vi "Encode String.vi"(7 "Prepend BOM (F)":bool, 8 "error in":errorcluster, 9 "Output Encoding (UTF-16LE)":T1=enum."UTF-16LE", 10 "Input Encoding (ANSI)":T1, 11 "String in":string) -> (0 "error out":errorcluster, 3 "String out":string)   [LabVIEW 2020, in "G-Unicode.lvlib"]
doc: "Encodes the text in <b>String</b> with the encoding specified by <b>Output Encoding</b>. The input String encoding is defined by <b>Input Encoding</b>. If Output Encoding is unicode (UTF-8 or UTF-16), the corresponding Byte Order Mark (BOM) can be prepended by setting <b>Prepend BOM</b> to TRUE.\n\nIf the input string encoding isn't known, Input Encoding can be set to Unknown to try and automatically detect the encoding method. Note that automatic encoding detection isn't 100% accurate, and it is recommended to set the encoding explicitly if it is known.\n\nSupported input/output encodings:\nANSI\nUTF-8\nUTF-16LE\nUTF-16BE"
uses:
  G-Unicode.lvlib
  Controls/String Encoding.ctl
  Private/Conversion/Polymorphic VIs/Text to UTF-8 (LabVIEW String).vi
  Private/Conversion/Polymorphic VIs/UTF-8 to Text (LabVIEW String).vi
  SubVIs/Byte Order Marks.vi
  Detect BOM.vi
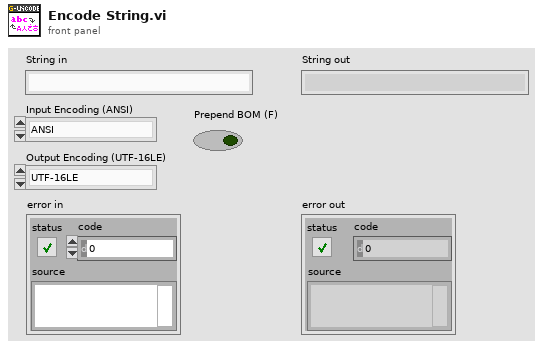
[diagram p1: front panel]
types:
  T1 = typedef "G-Unicode.lvlib/String Encoding.ctl" = enum16{"ANSI", "UTF-8", "UTF-16LE", "UTF-16BE", "Unknown"}
  T2 = typedef "G-Unicode.lvlib/Encoded UTF-8 String.ctl" = string
  T3 = typedef "G-Unicode.lvlib/Encoded UTF-16LE String.ctl" = string
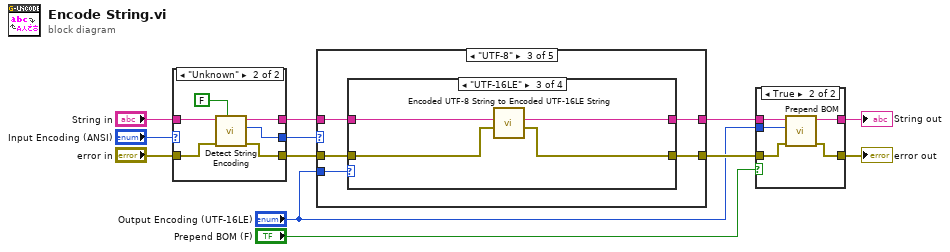
[diagram p0: block diagram]
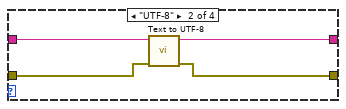
[diagram p5: hidden frame]
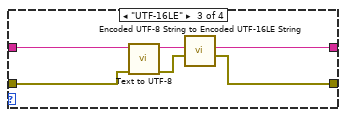
[diagram p6: hidden frame]
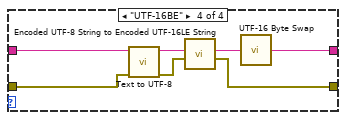
[diagram p7: hidden frame]
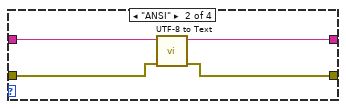
[diagram p9: hidden frame]
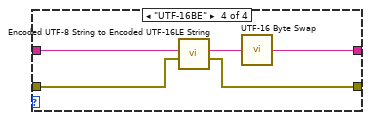
[diagram p10: hidden frame]
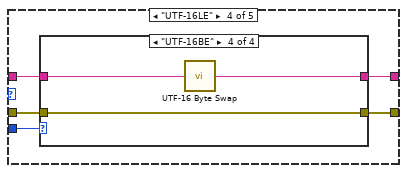
[diagram p11: hidden frame]
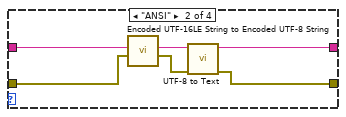
[diagram p13: hidden frame]
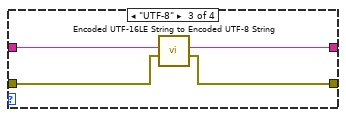
[diagram p14: hidden frame]
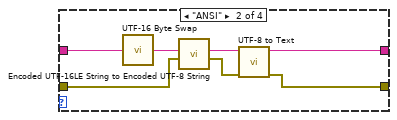
[diagram p16: hidden frame]
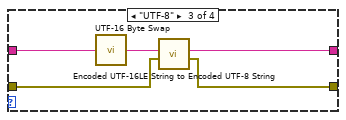
[diagram p17: hidden frame]
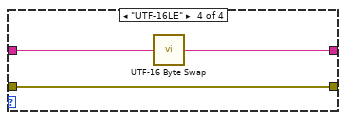
[diagram p18: hidden frame]
diagram:
  n1 = case shown="\"Unknown\"" "Input Encoding (ANSI)" {
    selector: "Input Encoding (ANSI)" -> [w13 _]
    tunnel: "String in" -> [w15 w21]
    tunnel: [w13 w20] -> w8
    tunnel: [w15 w19] -> w9
    tunnel: "error in" -> [w14 w16]
    tunnel: [w14 w17] -> w7
    frame Default {
    }
    frame "Unknown" {
      n2 = call "Detect String Encoding.vi"("Strip BOM (T)"=FALSE ("Remove BOM (T)"), "error in"=w16, "String"=w21) -> ("error out"=w17:errorcluster, "Encoding"=w20:T1, "String out"=w19:string)  [unwired: 6 in]
    }
  }
  n3 = case shown="\"UTF-8\"" w8 {
    tunnel: w9 -> [w23 w27 w50 w70 w90]
    tunnel: "Output Encoding (UTF-16LE)" -> [_ w24 w52 w72 w92]
    tunnel: w7 -> [w22 w26 w49 w69 w89]
    tunnel: [w23 w28 w51 w71 w91] -> w6
    tunnel: [w22 w25 w48 w68 w88] -> w4
    frame Default {
    }
    frame "ANSI" {
      n4 = case shown="Default" w24 {
        tunnel: [w30 w31 w38 w41] -> w28
        tunnel: w27 -> [w30 w34 w40 w47]
        tunnel: w26 -> [w29 w33 w37 w44]
        tunnel: [w29 w32 w35 w42] -> w25
        frame Default {
        }
        frame "UTF-8" {
          n5 = call-poly "Text to UTF-8.vi"("error in"=w33, "String"=w34) -> ("error out"=w32:errorcluster, "UTF-8 Encoded String"=w31:T2)  [unwired: 8 in]
        }
        frame "UTF-16LE" {
          n6 = call-poly "Text to UTF-8.vi"("error in"=w37, "String"=w40) -> ("error out"=w36:errorcluster, "UTF-8 Encoded String"=w39:T2)  [unwired: 8 in]
          n7 = call "Encoded UTF-8 String to Encoded UTF-16LE String.vi"("error in"=w36, "Encoded UTF-8 String"=w39) -> ("error out"=w35:errorcluster, "Encoded UTF-16LE String"=w38:T3)  [unwired: 8 in]
        }
        frame "UTF-16BE" {
          n8 = call-poly "Text to UTF-8.vi"("error in"=w44, "String"=w47) -> ("error out"=w43:errorcluster, "UTF-8 Encoded String"=w46:T2)  [unwired: 8 in]
          n9 = call "Encoded UTF-8 String to Encoded UTF-16LE String.vi"("error in"=w43, "Encoded UTF-8 String"=w46) -> ("error out"=w42:errorcluster, "Encoded UTF-16LE String"=w45:T3)  [unwired: 8 in]
          n10 = call "UTF-16 Byte Swap.vi"("String in"=w45) -> ("String out"=w41:string)
        }
      }
    }
    frame "UTF-8" {
      n11 = case shown="\"UTF-16LE\"" w52 {
        tunnel: [w54 w57 w62 w63] -> w51
        tunnel: w50 -> [w54 w58 w60 w65]
        tunnel: w49 -> [w53 w55 w59 w64]
        tunnel: [w53 w56 w61 w66] -> w48
        frame Default {
        }
        frame "ANSI" {
          n12 = call-poly "UTF-8 to Text.vi"("error in"=w55, "UTF-8 Encoded String"=w58) -> ("error out"=w56:errorcluster, "String"=w57:string)  [unwired: 8 in]
        }
        frame "UTF-16LE" {
          n13 = call "Encoded UTF-8 String to Encoded UTF-16LE String.vi"("error in"=w59, "Encoded UTF-8 String"=w60) -> ("error out"=w61:errorcluster, "Encoded UTF-16LE String"=w62:T3)  [unwired: 8 in]
        }
        frame "UTF-16BE" {
          n14 = call "Encoded UTF-8 String to Encoded UTF-16LE String.vi"("error in"=w64, "Encoded UTF-8 String"=w65) -> ("error out"=w66:errorcluster, "Encoded UTF-16LE String"=w67:T3)  [unwired: 8 in]
          n15 = call "UTF-16 Byte Swap.vi"("String in"=w67) -> ("String out"=w63:string)
        }
      }
    }
    frame "UTF-16LE" {
      n16 = case shown="\"UTF-16BE\"" w72 {
        tunnel: [w74 w80 w84 w86] -> w71
        tunnel: w70 -> [w74 w77 w83 w87]
        tunnel: w69 -> [w73 w75 w81 w85]
        tunnel: [w73 w79 w82 w85] -> w68
        frame Default {
        }
        frame "ANSI" {
          n17 = call "Encoded UTF-16LE String to Encoded UTF-8 String.vi"("error in"=w75, "Encoded UTF-16LE String"=w77) -> ("error out"=w76:errorcluster, "Encoded UTF-8 String"=w78:T2)  [unwired: 8 in]
          n18 = call-poly "UTF-8 to Text.vi"("error in"=w76, "UTF-8 Encoded String"=w78) -> ("error out"=w79:errorcluster, "String"=w80:string)  [unwired: 8 in]
        }
        frame "UTF-8" {
          n19 = call "Encoded UTF-16LE String to Encoded UTF-8 String.vi"("error in"=w81, "Encoded UTF-16LE String"=w83) -> ("error out"=w82:errorcluster, "Encoded UTF-8 String"=w84:T2)  [unwired: 8 in]
        }
        frame "UTF-16BE" {
          n20 = call "UTF-16 Byte Swap.vi"("String in"=w87) -> ("String out"=w86:string)
        }
      }
    }
    frame "UTF-16BE" {
      n21 = case shown="Default" w92 {
        tunnel: [w94 w101 w106 w108] -> w91
        tunnel: w90 -> [w94 w98 w105 w109]
        tunnel: w89 -> [w93 w96 w103 w107]
        tunnel: [w93 w100 w104 w107] -> w88
        frame Default {
        }
        frame "ANSI" {
          n22 = call "UTF-16 Byte Swap.vi"("String in"=w98) -> ("String out"=w95:string)
          n23 = call "Encoded UTF-16LE String to Encoded UTF-8 String.vi"("error in"=w96, "Encoded UTF-16LE String"=w95) -> ("error out"=w97:errorcluster, "Encoded UTF-8 String"=w99:T2)  [unwired: 8 in]
          n24 = call-poly "UTF-8 to Text.vi"("error in"=w97, "UTF-8 Encoded String"=w99) -> ("error out"=w100:errorcluster, "String"=w101:string)  [unwired: 8 in]
        }
        frame "UTF-8" {
          n25 = call "UTF-16 Byte Swap.vi"("String in"=w105) -> ("String out"=w102:string)
          n26 = call "Encoded UTF-16LE String to Encoded UTF-8 String.vi"("error in"=w103, "Encoded UTF-16LE String"=w102) -> ("error out"=w104:errorcluster, "Encoded UTF-8 String"=w106:T2)  [unwired: 8 in]
        }
        frame "UTF-16LE" {
          n27 = call "UTF-16 Byte Swap.vi"("String in"=w109) -> ("String out"=w108:string)
        }
      }
    }
  }
  n28 = case shown="True" "Prepend BOM (F)" {
    tunnel: w6 -> [w111 w116]
    tunnel: [w111 w115] -> w5
    tunnel: w4 -> [w110 w114]
    tunnel: [w110 w113] -> w3
    tunnel: "Output Encoding (UTF-16LE)" -> [_ w112]
    frame False {
    }
    frame True {
      n29 = call "Prepend BOM.vi"("error in"=w114, "Input Encoding (UTF-16LE)"=w112, "String"=w116) -> ("error out"=w113:errorcluster, "String with BOM"=w115:string)  [unwired: 7 in]
    }
  }
  "String out" <- w5
  "error out" <- w3
